vi "UMLEditor Main.vi"(1 "StartProject":string, 3 "StartTarget":string) -> ()   [LabVIEW 2020]
doc: "Main Open UML Modeller VI"
uses:
  <resource>/Framework/Providers/Open_GDS/UML/UMLEditor/UMLEditor statesType.ctl
  <resource>/Framework/Providers/Open_GDS/UML/UMLEditor/UMLEditor LocalVariablesType.ctl
  <resource>/Framework/Providers/Open_GDS/UML/Graphics_class/Graphics.lvclass
  <resource>/Framework/Providers/Open_GDS/UML/Grid_class/Grid.lvclass
  <resource>/Framework/Providers/Open_GDS/UML/UMLEditor/UMLEditor tooltype.ctl
  <resource>/Framework/Providers/Open_GDS/UML/UMLEditor/UMLEditor_DiagramInfo.ctl
  <resource>/Framework/Providers/Open_GDS/UML/Graph_class/Graph.lvclass
  <resource>/Framework/Providers/Open_GDS/UML/General/Point/Point Point2D.ctl
  <resource>/Framework/Providers/Open_GDS/UML/General/Rectangle/Rectangle Rectangle2D.ctl
  <resource>/Framework/Providers/Open_GDS/UML/AbstractEdge_class/AbstractEdge.lvclass
  <resource>/Framework/Providers/Open_GDS/UML/UMLEditor/UMLEditor ExportType.ctl
  <resource>/Framework/Providers/Open_GDS/UML/UMLEditor/UMLEditor FlattenCommandType.ctl
  <resource>/Framework/Providers/Open_GDS/UML/UMLEditor/UMLEditor ExecuteCommandType.ctl
  <resource>/Framework/Providers/Open_GDS/UML/ContextHelp/ContextHelp_EventType.ctl
  <resource>/Framework/Providers/Open_GDS/UML/AbstractNode_class/AbstractNode.lvclass
  <resource>/Framework/Providers/Open_GDS/UML/UMLEditor/UMLEditor_HotSpotData.ctl
  <resource>/Framework/Providers/Open_GDS/UML/UMLEditor/UMLEditor_HotSpotType.ctl
  <resource>/Framework/Providers/Open_GDS/UML/UmlEditor_class/EventData.ctl
  <resource>/Framework/Providers/Open_GDS/UML/ClassDiagramGraph_class/ClassDiagramGraph.lvclass
  C:/Program Files (x86)/National Instruments/LabVIEW 2020/resource/Framework/Providers/Open_GDS/UML/Graph_class/Graph.lvclass
  <resource>/Framework/Providers/Open_GDS/UML/DqmhModuleDiagramGraph_class/DqmhModuleDiagramGraph.lvclass
  <resource>/Framework/Providers/Open_GDS/UML/SequenceDiagramGraph_class/SequenceDiagramGraph.lvclass
  <resource>/Framework/Providers/Open_GDS/UML/StateDiagramGraph_class/StateDiagramGraph.lvclass
  <resource>/Framework/Providers/Open_GDS/UML/UseCaseDiagramGraph_class/UseCaseDiagramGraph.lvclass
  <resource>/Framework/Providers/Open_GDS/UML/UMLEditor/UMLEditor_Cursortype.ctl
  <resource>/Framework/Providers/Open_GDS/UML/UMLEditor/UMLEditor MenuActionType.ctl
  <resource>/Framework/Providers/Open_GDS/UML/Graphics_class/LvFontType.ctl
  <resource>/Framework/Providers/Open_GDS/UML/Graphics_class/FontType.ctl
  <resource>/Framework/Providers/Open_GDS/UML/UMLEditor/UMLEditor BusyDialogAction.ctl
  <resource>/Framework/Providers/Open_GDS/UML/UMLEditor/UMLEditor_StoredPathes.ctl
  <resource>/Framework/Providers/Open_GDS/ClassProviders/Common/File/File_StoredPathesActions.ctl
  <resource>/Framework/Providers/Open_GDS/UML/ContextHelp/ContextHelp_HelpTexts.ctl
  <resource>/Framework/Providers/Open_GDS/UML/GeneralPathEdge_class/GeneralPathEdge.lvclass
  C:/Program Files (x86)/National Instruments/LabVIEW 2020/resource/Framework/Providers/Open_GDS/UML/AbstractEdge_class/AbstractEdge.lvclass
  <resource>/Framework/Providers/Open_GDS/UML/ClassNode_class/ClassNode.lvclass
  C:/Program Files (x86)/National Instruments/LabVIEW 2020/resource/Framework/Providers/Open_GDS/UML/AbstractNode_class/AbstractNode.lvclass
  <vilib>/event_ctls.llb/eventvkey.ctl
  <resource>/Framework/Providers/Open_GDS/UML/Graph_class/SaveTypes.ctl
  <resource>/Framework/Providers/Open_GDS/UML/UMLEditor/UMLEditor_DiagramType.ctl
  <resource>/Framework/Providers/Open_GDS/UML/ClassNode_class/ExternalSetTypes.ctl
  <resource>/Framework/Providers/Open_GDS/UML/StateDiagramGraph_class/private/StateDiagramData.ctl
  <resource>/Framework/Providers/Open_GDS/UML/StateDiagramGraph_class/private/ViPathShowOption.ctl
  <resource>/Framework/Providers/Open_GDS/UML/UMLEditor/UMLEditor ClipBoardActionType.ctl
  <resource>/Framework/Providers/Open_GDS/UML/RectangularNode_class/RectangularNode.lvclass
  <resource>/Framework/Providers/Open_GDS/UML/ReversedEngineering/private/ReversedEngineering SyncUmlFromCodeActions.ctl
  <resource>/Framework/Providers/Open_GDS/ClassProviders/Common/CommonVIs/CommonVIs_StereoType.ctl
  Instance           1 22Saved   UMLEditor Main .vi
  Instance           2 22Saved   UMLEditor Main .vi
  <resource>/Framework/Providers/Open_GDS/ClassProviders/Provider_BaseClassInterface/ClassReader_class/ClassReader.lvclass
  <resource>/Framework/Providers/Open_GDS/UML/UMLEditor/UMLEditor ToolButtonsAction.ctl
  <resource>/Framework/Providers/Open_GDS/UML/UmlEditor_class/UmlEditor.lvclass
  <vilib>/Utility/cursorutil.llb/Set Cursor (Icon Pict).vi
panel:
  in  "GraphButtons":T1(radio)=enum."2" caption="Radio Buttons"
  out "SearchString":string caption="Search"
  in  "open":bool
  in  "close":bool
  in  "Diagram":u16(ring) items=["Class Diagram: 22.uml"]
  out "ProductPicture":picture
  out "Time":i32=21
  out "PictureMenuEvent":string
  out "RevHistory":bool
  in  "Help":bool
  in  "DragAndDropPath":path
  in  "ClassAggregationDialog":T2
  out "Picture":picture
  out "error out":errorcluster
  in  "Project":u16(ring) items=["GDS_Example_022.lvproj"]
  in  "Help":bool=TRUE
  in  "Target":u16(ring) items=["My Computer"]
  out "StatusBar":string
  in  "Sync":bool
  # "Class aggregation"
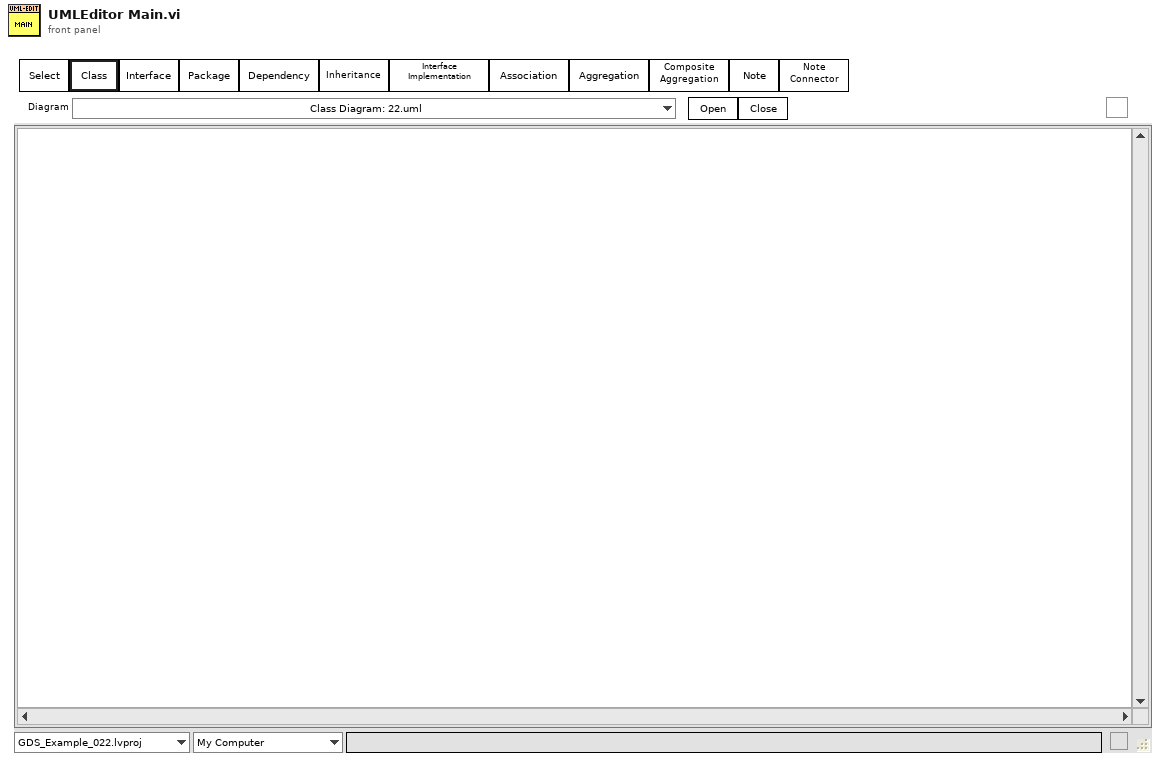
[diagram p1: front panel]
types:
  T1 = enum32{"1", "2", "3", "4", "5", "6", "7", "8", "9", "10", "11", "12", "13"}
  T2 = cluster{"AddAttribute":bool, "Don'tAddAttribute":bool, "Close":bool, "Text":string}
  T3 = typedef "UMLEditor MenuActionType.ctl" = enum16{"EnableSave", "EnablePaste", "DisablePaste", "DiableSave", "AddRecentFile", "disablePropDel", "enablePropDel", "enablePropDisDel", "diasbleClassRel", "enableClassRel", "Class", "State", "Other", "EnableXMI", "DisableXMI", "EnableCopy", "DisableCopy"}
  T4 = typedef "UMLEditor_Cursortype.ctl" = enum16{"Arrow", "Move", "Finger", "Wait", "NS", "WE", "NESW", "NWSE"}
  T5 = typedef "UMLEditor LocalVariablesType.ctl" = cluster{"state":T6, "graphics":refnum<class "Graphics.lvclass">, "grid":refnum<class "Grid.lvclass">, "toolType":T7, "diagramIndex":i32, "diagrams":T8[], "zoom":dbl, "hideGrid":bool, "lastMousePoint":T9, "rubberBandStart":T9, "dragStartPoint":T9, "dragStartBounds":T10, "gridColor":u32, "gridSize":dbl, "CONNECT_THRESHOLD":i32, "selected":T7, "selectedEdge":refnum<class "AbstractEdge.lvclass">, "butDwn":bool, "lastPress":u32, "modified":bool, "offset":T9, "menu":refnum<k9>, "file":path, "saveAs":bool, "newSelected":bool, "exportype":T11, "quit":bool, "revHistory":cluster{"rev":string, "text":string}[], "FlattenCommandSettings":T12, "PopUpMessageEvent":T14, "ResizePanelInProgress":bool, "NodesBounds":T10, "ToolHelp":bool, "ViRef":refnum<vi>, "FP_CtrlEnterEvents":refnum<event-registration>, "SelectedNodes":refnum<class "AbstractNode.lvclass">[], "mouse":refnum<k1>, "RevPlugInPath":path, "Action":string, "KeyPressTime":u32, "ObjectHotspots":T15[], "HotSpotCursor":bool, "HotSpotFunction":T16, "Don'tDeleteChildren":bool, "ShiftDown":bool, "CtrlDown":bool, "HotSpotNode":refnum<class "AbstractNode.lvclass">, "Sync":bool, "SyncTime":u32, "ForceSyncNow":bool, "LastSync":timestamp, "XMI_Import":bool, "Event":refnum<event-registration>}
  T6 = typedef "UMLEditor statesType.ctl" = enum16{"Idle", "CheckLicense", "revHistory", "Init", "Init2", "EditSelected", "RemoveSelected", "PaintComponent", "ChangeZoom", "ChangeGridSize", "Open", "Close", "Save", "ExportPicture", "Export", "Repaint", "Error", "Exit", "QUIT", "CreateScript", "ExecuteScript", "ClassReversedEngineering", "PlugInReverseEngineering", "StateReversedEngineering", "AutoPlace", "ExecuteCommand", "OpenClass", "SyncAll", "StraightenAssociation", "Copy", "Paste", "AddNodeFromProjectTree", "AddNodeFromProjectTree+SyncAll", "PanAndRepaint", "Init3", "CopyPaste", "ApplyDesignPattern", "AnalyseViInStateDiagram", "AutoSync"}
  T7 = typedef "UMLEditor tooltype.ctl" = enum16{"None", "Node", "Edge"}
  T8 = typedef "UMLEditor_DiagramInfo.ctl" = cluster{"name":string, "diagramType":string, "unsaved":bool, "graph":refnum<class "Graph.lvclass">, "saveDir":path}
  T9 = typedef "Point Point2D.ctl" = cluster{"x":dbl, "y":dbl}
  T10 = typedef "Rectangle Rectangle2D.ctl" = cluster{"x":dbl, "y":dbl, "width":dbl, "height":dbl}
  T11 = typedef "UMLEditor ExportType.ctl" = enum16{"None", "Printer", "png", "jpg", "roseUML"}
  T12 = typedef "UMLEditor FlattenCommandType.ctl" = cluster{"Command":T13, "CommandData":variant}
  T13 = typedef "UMLEditor ExecuteCommandType.ctl" = enum16{"SyncUmlFromCode", "SyncCodeFromUML", "OpenClass", "OpenFile", "CreateClass", "CreateVI", "OpenClassAttribute", "LocateInProject", "GraphExecute"}
  T14 = typedef "ContextHelp_EventType.ctl" = refnum<user-event>
  T15 = typedef "UMLEditor_HotSpotData.ctl" = cluster{"Node":refnum<class "AbstractNode.lvclass">, "HotSpot":T9, "Function":T16}
  T16 = typedef "UMLEditor_HotSpotType.ctl" = enum16{"N", "NE", "E", "SE", "S", "SW", "W", "NW", "Expand", "Collaps"}
  T17 = typedef "UMLEditor ToolButtonsAction.ctl" = enum16{"SelectSelect", "SetReferneces"}
  T18 = typedef "Graphics.lvclass/FontType.ctl" = cluster{"Font Name:":string, "Size":i16, "Strikeout?":bool, "Italic?":bool, "Underline?":bool, "Outline?":bool, "Shadow?":bool, "Bold?":bool}
  T19 = enum16{"CreateAggregation", "DeleteAggregation", "SetReferneces", "HideCluster", "GetStatus"}
  T20 = typedef "Graphics.lvclass/LvFontType.ctl" = enum16{"User-specified Font", "Application Font", "System Font", "Dialog Font"}
  T21 = typedef "UMLEditor_StoredPathes.ctl" = enum16{"LastSearchPath", "QueuedArrayStateVI", "ClassBasePath", "ViTemplatePath", "ApplicationTemplatePath", "IniFilePath", "WizDir", "RevPlugInPath"}
  T22 = typedef "UMLEditor BusyDialogAction.ctl" = enum16{"Initialize", "Open(VIs)", "Open(i)", "Send_I-Value", "SendStatusMessage", "GetBusyDialogStatus", "Close", "Quit"}
  T23 = enum16{"SetPopUpEventTask", "GetStatus", "SetOpenState", "SetDialogCaller", "SetToolHelp"}
  T24 = typedef "File_StoredPathesActions.ctl" = enum16{"Get Path", "Set Path", "Delete Path", "Clear All Paths"}
  T25 = typedef "ContextHelp_HelpTexts.ctl" = enum16{"None(Hide)", "Default", "Help", "Welcome", "GettingStarted", "ClassDiagram_Help", "SequenceDiagram_Help", "UseCaseDiagram_Help", "BSelect", "BClass", "BInterface", "BPackage", "BNote", "BDependency", "BInheritance", "BInterfaceImplementation", "BAssociation", "BAggregation", "BCompAggregation", "BNoteConnector", "BObject", "BActionBar", "BCall", "BSystem", "BActor", "BUseCase", "BGeneralization", "BIncludes", "BExtends", "BUseCaseDiagramAssociation", "ClassRelationshipEdge editDialog_Bent Style", "ClassRelationshipEdge editDialog_RelationType", "ClassRelationshipEdge editDialog_Reverse association", "ClassRelationshipEdge editDialog_Start label", "ClassRelationshipEdge editDialog_Middle label", "ClassRelationshipEdge editDialog_End label", "UMLEditor reversedEngineering_Pathes", "ReversedEngineering StateReverseDialog_Help", "ReversedEngineering StateQueuedSettings_Help", "UMLEditor reversedEngineering_AddTopVIs", "UMLEditor reversedEngineering_AddClasses", "UMLEditor reversedEngineering_AddDirs", "UMLEditor reversedEngineering_Recursively", "UMLEditor reversedEngineering_Remove", "UMLEditor reversedEngineering_ClearList", "UMLEditor reversedEngineering_HideSubAss", "UMLEditor reversedEngineering_CreateTypes", "UMLEditor reversedEngineering_OnlyInheritance", "UMLEditor reversedEngineering_CreateApplication", "UMLEditor reversedEngineering_OK", "UMLEditor reversedEngineering_Cancel", "UMLEditor reversedEngineering_Help", "UMLEditor createWizardScriptFile_ScriptfilePath", "UMLEditor createWizardScriptFile_ClassPath", "UMLEditor createWizardScriptFile_Use", "UMLEditor createWizardScriptFile_PrivateDirName", "UMLEditor createWizardScriptFile_DirAppend", "UMLEditor createWizardScriptFile_Separator Character", "UMLEditor createWizardScriptFile_OK", "UMLEditor createWizardScriptFile_Cancel", "UMLEditor createWizardScriptFile_Help", "ClassNode editDialog_Class Name", "InterfaceNode editDialog_Class Name", "ClassNode editDialog_Attribute", "ClassNode editDialog_Methods", "InterfaceNode editDialog_Methods", "ClassNode editDialog_connection", "InterfaceNode editDialog_connection", "ClassNode editDialog_StereoType", "ClassNode editDialog_ShowAttrib", "ClassNode editDialog_ShowMethods", "ClassNode editDialog_ClassPath", "ClassNode editDialog_AddAttribute", "ClassNode editDialog_AddMethod", "InterfaceNode editDialog_AddMethod", "ClassNode AttributeGuide_AttributeName", "ClassNode AttributeGuide_Array?", "ClassNode AttributeGuide_Data Type", "ClassNode AttributeGuide_RefName", "ClassNode AttributeGuide_Preview", "ClassNode AttributeGuide_OK", "ClassNode AttributeGuide_Cancel", "ClassNode MethodGuide_Visibility", "ClassNode MethodGuide_Method Name", "ClassNode MethodGuide_Preview", "ClassNode MethodGuide_OK", "ClassNode MethodGuide_Cancel", "CallNode EditCallProperties_AllButtons", "ObjectNode EditObjectlProperties_AllButtons", "ActorNode EditActorProperties_AllButtons", "UseCaseRelationshipNode EditUseCaselProperties_AllButtons", "UseCaseNode EditUseCaselProperties_AllButtons", "SystemNode EditSystemProperties_AllButtons", "ReversedEngineering UpdateAttributes_AllButtons", "StateNode editDialog_AllButtons", "StateTransition editDialog_AllButtons", "ArrangeNodes Main_Picture", "ArrangeNodes Main_Zoom", "ArrangeNodes Main_Auto Zoom", "ArrangeNodes Main_shorten", "ArrangeNodes Main_Min Length", "ArrangeNodes Main_Max Length", "ArrangeNodes Main_increase", "ArrangeNodes Main_decrease", "ArrangeNodes Main_Shake", "ArrangeNodes Main", "BState", "BInitialState", "BFinalState", "BStateTransition", "StateDiagram_Help", "StateDiagram_PropertiesAllButtons", "ReversedEngineering StateReverseDialog_ClearStates", "ReversedEngineering StateReverseDialog_UseQueuedStateMachines", "ReversedEngineering StateReverseDialog_QueuedSettings", "ReversedEngineering StateReverseDialog_SearchForVIs", "ReversedEngineering StateReverseDialog_SearchCriteria", "OptionsDialog_ClassBasePath", "OptionsDialog_VIPath", "OptionsDialog_ApplicationPath", "OptionsDialog_WizDir", "OptionsDialog_IniFilePath", "OptionsDialog_DefineColors", "OptionsDialog_Help", "OptionsDialog_CreateTypes", "ClassRelationshipEdge editDialog_SplitWire"}
  T26 = typedef "Graph.lvclass/SaveTypes.ctl" = enum16{"Normal", "XMI"}
  T27 = typedef "UMLEditor_DiagramType.ctl" = string
  T28 = typedef "ClassNode.lvclass/ExternalSetTypes.ctl" = enum16{"Name", "Attributes", "Methods", "Position", "ShowMethods", "ShowAttributes", "ClassPath"}
  T29 = typedef "StateDiagramGraph.lvclass/StateDiagramData.ctl" = cluster{"VI-Path":path, "ShowOption":T30}
  T30 = typedef "StateDiagramGraph.lvclass/ViPathShowOption.ctl" = enum16{"Don't Show", "Show Relative Path", "Show Absolute Path"}
  T31 = typedef "UMLEditor ClipBoardActionType.ctl" = enum16{"Init", "EmptyClipBoard", "InsertToClipBoard", "PasteContentAtPos"}
  T32 = enum16{"Left Button", "Center Button", "Right Button", "Window Close"}
  T33 = typedef "ReversedEngineering SyncUmlFromCodeActions.ctl" = enum16{"GetAttributes&MethodsFromCode", "GetAll"}
  T34 = typedef "CommonVIs_StereoType.ctl" = enum16{"None", "TYPE", "ENUM", "ABSTRACT", "ACTOR", "GUI", "SINGLETON", "SIGNAL", "BOUNDARY", "ENTITY", "CONTROL", "LEGACY", "APPLICATION", "VI", "LVLIB", "INTERFACE"}
  T35 = enum8{"Enabled", "Disabled", "Disabled and Grayed Out"}
  T36 = typedef "Graph.lvclass/ToolbarButtonType.ctl" = cluster{"Text":string, "Type":T7}
  T37 = cluster{"startNode":refnum<class "AbstractNode.lvclass">, "endNode":refnum<class "AbstractNode.lvclass">}
  T38 = typedef "ContextHelp_ShowType.ctl" = cluster{"Header":string, "Picture":picture, "Text":string}
  T39 = typedef "LVPoint32TypeDef.ctl" = cluster{"Horizontal":i32, "Vertical":i32}
  T40 = typedef "eventsource.ctl" = u32
  T41 = typedef "LVMouseTypeDef.ctl" = cluster{"Mouse Position":cluster{"X":i32, "Y":i32}, "Mouse Modifiers":cluster{"Button Down":bool, "Shift Mod":bool, "Menu Mod":bool, "Option Mod":bool}}
  T42 = typedef "LVBoundsTypeDef.ctl" = cluster{"Width":u32, "Height":u32}
  T43 = typedef "LVPointTypeDef.ctl" = cluster{"Horizontal":i16, "Vertical":i16}
  T44 = typedef "UMLEditor toolsType.ctl" = enum16{"CD_Select", "CD_Class", "CD_Interface", "CD_Package", "CD_Note", "CD_Dependency", "CD_Inheritance", "CD_InterfaceImp", "CD_Association", "CD_Aggregation", "CD_Composite", "CD_NoteConn", "SQD_Select", "SQD_Object", "SQD_ActionBar", "SQD_Note", "SQD_Call", "SQD_NoteConn", "UD_Select", "UD_System", "UD_Actor", "UD_UseCase", "UD_Note", "UD_Assoiciation", "UD_Generalization", "UD_GeneralizationIncludes", "UD_GeneralizationExtends", "UD_Realization", "UD_Relationship", "UD_NoteEdge", "STD_Select", "STD_State", "STD_InitailState", "STD_FinalState", "STD_ChoiseState", "STD_StateTransation", "STD_Note", "STD_NoteEdge", "DM_Select", "DM_VI", "DM_Module", "DM_Request", "DM_RequestWait", "DM_Roundtrip", "DM_Broadcast", "DM_Note", "DM_NoteEdge"}
  T45 = cluster{"Shift":bool, "Ctrl":bool, "Alt":bool, "Cmd":bool, "Opt":bool}
  T46 = typedef "UMLEditor EditorActionType.ctl" = enum16{"NoAction", "Repaint", "ExecuteCommand"}
  T47 = typedef "eventvkey.ctl" = enum16{"ASCII", "Enter", "Return", "Shift", "Ctrl", "Alt", "Cmd", "Opt", "Caps", "NumLock", "Clear", "Break", "Up", "Down", "Left", "Right", "Insert", "Delete", "Home", "End", "PageUp", "PageDown", "Escape", "Help", "Pause", "ScrollLock", "F1", "F2", "F3", "F4", "F5", "F6", "F7", "F8", "F9", "F10", "F11", "F12", "F13", "F14", "F15", "F16", "F17", "F18", "F19", "F20", "F21", "F22", "F23", "F24", "Play", "VolumeUp", "VolumeDown", "Mute", "Two Byte Char"}
  T48 = typedef "lveventtype.ctl" = enum32{"Null", "Timeout", "Annotation Menu Selection", "Annotation Menu Selection?", "App Instance Close", "App Instance Close?", "Autoscale Range Change", "Bookmark Info Change", "Cell Edit", "Cell Edit?", "Cursor Grab", "Cursor Grab?", "Cursor Menu Selection", "Cursor Menu Selection?", "Cursor Move", "Cursor Release", "Data Change", "Direction Change", "Display State Change", "Drag Ended", "Drag Enter", "Drag Leave", "Drag Over", "Drag Source Update", "Drag Starting", "Drag Starting?", "Drop", "Exec State Change", "Key Down", "Key Down?", "Key Repeat", "Key Repeat?", "Key Up", "Listbox Double Click", "Menu Activation?", "Menu Selection (App)", "Menu Selection? (App)", "Menu Selection (User)", "Mouse Down", "Mouse Down?", "Mouse Enter", "Mouse Leave", "Mouse Move", "Mouse Up", "Mouse Wheel", "NI Security User Change (App)", "Pane Size", "Panel Close", "Panel Close?", "Panel Resize", "Plot Attribute Change", "Scale Range Change", "Shortcut Menu Activation?", "Shortcut Menu Selection (App)", "Shortcut Menu Selection? (App)", "Shortcut Menu Selection (User)", "Tree Double Click", "Tree Drag", "Tree Drag?", "Tree Drop", "Tree Drop?", "Tree Item Close", "Tree Item Close?", "Tree Item Open", "Tree Item Open?", "User Event", "Value Change"}
  T49 = enum32{"existing file", "new file", "new or existing file", "existing dir", "new dir", "new or existing dir", "existing file (use LLBs)", "new file (use LLBs)", "new or existing file (use LLBs)", "new or existing file or directory (use LLBs)"}
  T50 = cluster{"button 1":bool, "button 2":bool, "button 3":bool, "button 4":bool}
  T51 = cluster{"Horizontal":i32, "Vertical":i32, "Scrolling":i32}
  T52 = typedef "LVRectTypeDef.ctl" = cluster{"Left":i16, "Top":i16, "Right":i16, "Bottom":i16}
  T53 = enum32{"Invalid", "Standard", "Closed", "Hidden", "Minimized", "Maximized"}
  T54 = typedef "AbstractNode.lvclass/NodeConnectionStatsType.ctl" = enum16{"NA", "Connect", "DisConnect"}
  T55 = typedef "Librarian File Info Out.ctl" = cluster{"creation date":u32, "last mod date":u32, "type":string, "creator":string, "LV version":i32, "size":i32, "top level":bool}
  T56 = typedef "Graph.lvclass/diagramType.ctl" = enum16{"None", "Class", "Sequency", "State", "UseCase"}
  T57 = typedef "DesignPatterns_Node.ctl" = cluster{"ID":string, "Type":T58, "Name":string, "Stereotype":string, "X":i32, "Y":i32, "TypeSpecificData":variant}
  T58 = typedef "DesignPatterns_NodeType.ctl" = enum16{"Class", "Interface", "Note", "Package"}
  T59 = typedef "DesignPatterns_Link.ctl" = cluster{"ID":string, "Type":T60, "Name":string, "StartText":string, "EndText":string, "From":string, "To":string, "BendStyle":string, "StartOffset":i32, "EndOffset":i32}
  T60 = typedef "DesignPatterns_LinkType.ctl" = enum16{"Dependency", "Inheritance", "Interface", "Association", "Aggregation", "CompositeAggregation"}
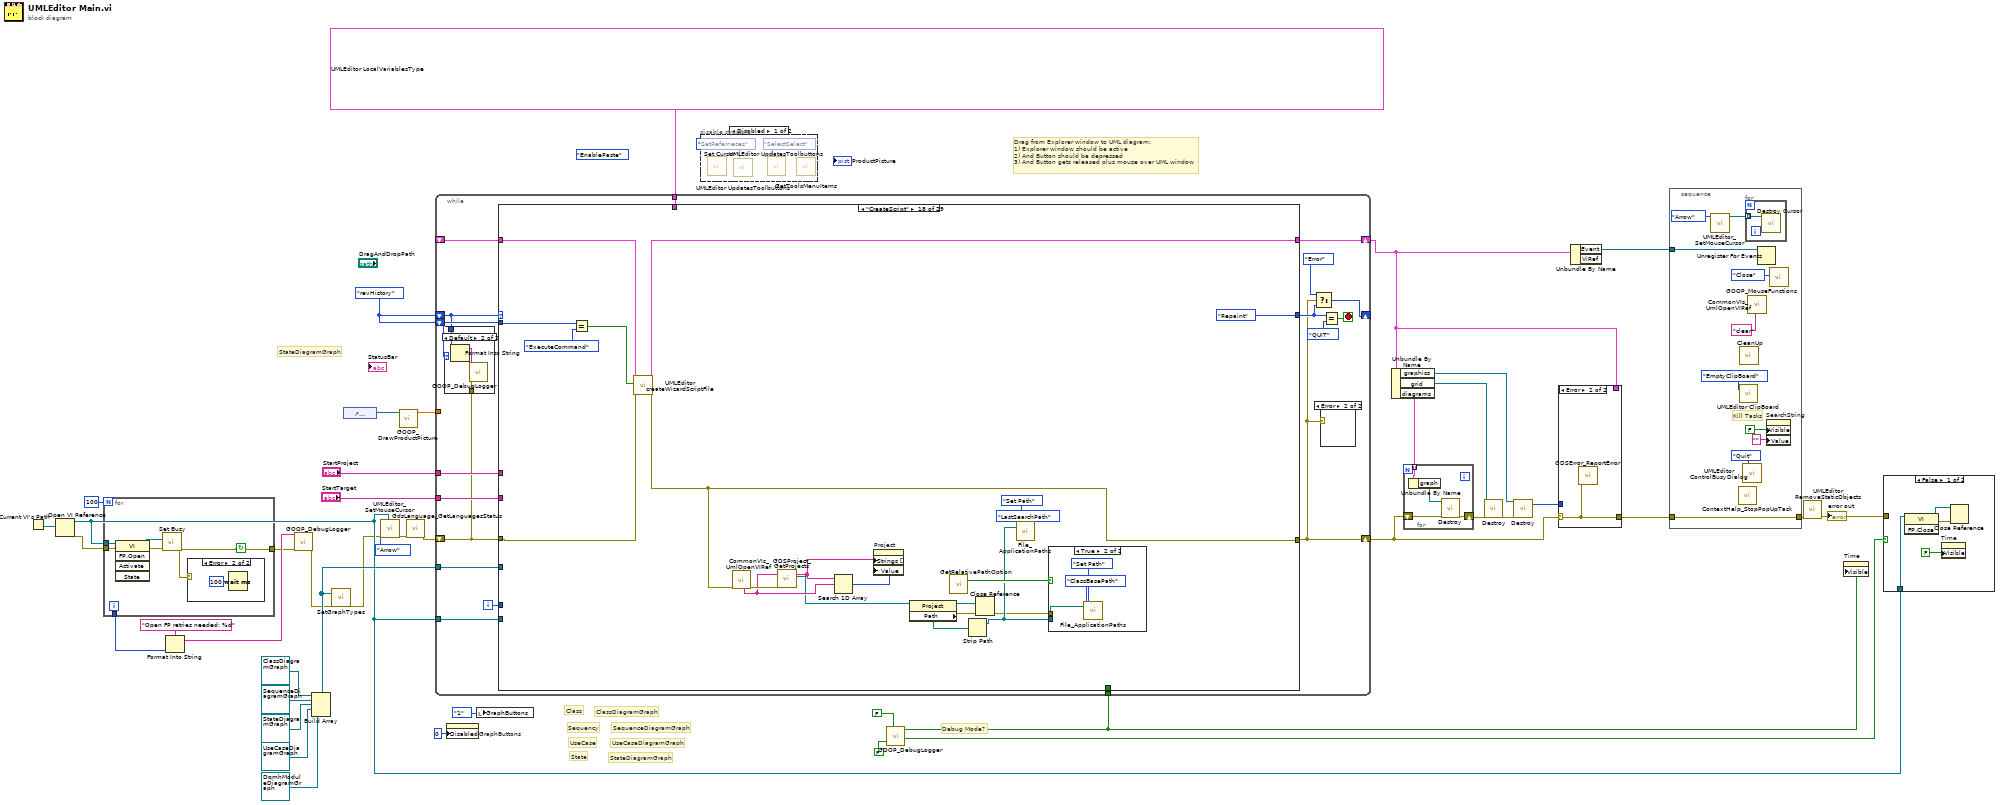
[diagram p0: block diagram]
diagram:
  (unwired) UMLEditor_MenuActionType."EnablePaste" ("menuAction")
  w37 = UMLEditor_statesType."revHistory" ("state")
  # "StateDiagramGraph"
  # "SequenceDiagramGraph"
  # "UseCaseDiagramGraph"
  # "State"
  # "UseCase"
  # "Sequency"
  # "ClassDiagramGraph"
  # "Class"
  # "StateDiagramGraph"
  # "Debug Mode?"
  # "Drag from Explorer window to UML diagram:\n1) Explorer window should be active\n2) And Button should be depressed\n3) And Button gets released plus mouse over UML window"
  n1 = Current VI's Path() -> (path=w34:path)
  n2 = Open VI Reference(vi path=w34) -> (vi reference=w9:refnum<vi>, error out=w8:errorcluster)  [unwired: 1 in, 4 out]
  n3 = for {
    N: 100 -> [_]
    tunnel: w9 -> [w49]
    tunnel: w8 -> [w48]
    tunnel: [w45] -> w3
    tunnel: [w44] -> w6
    i -> [w44]
    stop <- w45 continue-if-true
    n4 = invoke class="VI" method="FP.Open"(reference=w49, error in=w48) -> (reference out=w46:refnum<vi>, error out=w47:errorcluster)  [unwired: 3 in, 3 out]
    n5 = call <vilib>:"Set Busy.vi"("error in (no error)"=w47, "VI reference (current VI)"=w46) -> ("error out"=w45:errorcluster)  [unwired: 8 in, 1 out]
    n6 = case shown="Error" w45 {
      frame No Error {
      }
      frame Error {
        n7 = Wait (ms)(milliseconds to wait=u32 100) -> ()  [unwired: 1 out]
      }
    }
  }
  n8 = Format Into String(format string="Open FP retries needed: %d", w6) -> (resulting string=w4:string)  [unwired: 2 in, 1 out]
  n9 = call <resource>:"GOOP_DebugLogger.vi"("error in (no error)"=w3, "State"=w4) -> ("error out"=w2:errorcluster)  [unwired: 7 in, 2 out]
  n10 = Build Array(refnum<class "ClassDiagramGraph.lvclass"> refnum ("ClassDiagramGraph.lvclass"), refnum<class "SequenceDiagramGraph.lvclass"> refnum ("SequenceDiagramGraph.lvclass"), refnum<class "StateDiagramGraph.lvclass"> refnum ("StateDiagramGraph.lvclass"), refnum<class "UseCaseDiagramGraph.lvclass"> refnum ("UseCaseDiagramGraph.lvclass"), refnum<class "DqmhModuleDiagramGraph.lvclass"> refnum ("DqmhModuleDiagramGraph")) -> (w15:refnum<class "Graph.lvclass">[])
  n11 = call <resource>:"SetGraphTypes.vi"("GraphTypes"=w15, "error in (no error)"=w2) -> ("error out"=w1:errorcluster)  [unwired: 17 in]
  n12 = control-ref of="ProductPicture"() -> (w27:refnum<vi>)
  n13 = call <resource>:"UMLEditor_SetMouseCursor.vi"("ViRefToActOn"=w9, "error in (no error)"=w1, "CursorType"=UMLEditor_Cursortype."Arrow") -> ("error out"=w14:errorcluster)  [unwired: 7 in, 1 out]
  n14 = call <resource>:"GOOP_DrawProductPicture.vi"("ProductPictureControl"=w27) -> ("Zoom Factor"=w26:sgl)  [unwired: 10 in]
  n15 = call <resource>:"GdsLanguage_GetLanguagesStatus.vi"("error in (no error)"=w14) -> ("error out"=w32:errorcluster)  [unwired: 18 out]
  n16 = property on="GraphButtons" class="RadioBtnsControl (strict)"("Disabled"=u8 0) -> ()  [unwired: 2 in, 2 out]
  n17 = local write "GraphButtons"(T1."1" ("GraphButtons")) -> ()
  n18 = disable-structure shown="Disabled" {
    frame Disabled {
      n19 = call-poly <vilib>:"Set Cursor.vi"() -> ()  [unwired: 10 in, 2 out]
      n20 = call <resource>:"UMLEditor UpdatesToolbuttons.vi"("Action(SelectSelect)"=UMLEditor_ToolButtonsAction."SetReferneces") -> ()  [unwired: 5 in, 14 out]
      n21 = call <resource>:"UMLEditor UpdatesToolbuttons.vi"("Action(SelectSelect)"=UMLEditor_ToolButtonsAction."SelectSelect") -> ()  [unwired: 5 in, 14 out]
      n22 = call-dynamic "GetToolsMenuItems.vi"() -> ()  [unwired: 17 in, 3 out]
    }
    frame Enabled {
    }
  }
  n23 = call <resource>:"GOOP_DebugLogger.vi"("ActivateDon'tCloseVI"=FALSE ("ActivateDebugging"), "ActivateDebugging"=FALSE) -> ("Don'tCloseVI"=w24:bool, "Debugging"=w25:bool)  [unwired: 7 in, 1 out]
  n24 = while {
    shift-right: [w53] -> _
    shift-left: w37 -> [w58]
    shift-right: [w60] -> w28
    shift-left: w32 -> [w55]
    shift-right: [w67] -> w31
    shift-left: _ -> [w66]
    tunnel: T5 {"state"=enum."Idle", "graphics"=refnum, "grid"=refnum, "toolType"=enum."None", "diagramIndex"=0, "diagrams"=[], "zoom"=0.0, "hideGrid"=FALSE, "lastMousePoint"={"x"=0.0, "y"=0.0}, "rubberBandStart"={"x"=0.0, "y"=0.0}, "dragStartPoint"={"x"=0.0, "y"=0.0}, "dragStartBounds"={"x"=0.0, "y"=0.0, "width"=0.0, "height"=0.0}, "gridColor"=0, "gridSize"=0.0, "CONNECT_THRESHOLD"=0, "selected"=enum."None", "selectedEdge"=refnum, "butDwn"=FALSE, "lastPress"=0, "modified"=FALSE, "offset"={"x"=0.0, "y"=0.0}, "menu"=refnum, "file"=path "", "saveAs"=FALSE, "newSelected"=FALSE, "exportype"=enum."None", "quit"=FALSE, "revHistory"=[], "FlattenCommandSettings"={"Command"=enum."SyncUmlFromCode", "CommandData"=variant}, "PopUpMessageEvent"=refnum, "ResizePanelInProgress"=FALSE, "NodesBounds"={"x"=0.0, "y"=0.0, "width"=0.0, "height"=0.0}, "ToolHelp"=FALSE, "ViRef"=refnum, "FP_CtrlEnterEvents"=refnum, "SelectedNodes"=[], "mouse"=refnum, "RevPlugInPath"=path "", "Action"="", "KeyPressTime"=0, "ObjectHotspots"=[], "HotSpotCursor"=FALSE, "HotSpotFunction"=enum."N", "Don'tDeleteChildren"=FALSE, "ShiftDown"=FALSE, "CtrlDown"=FALSE, "HotSpotNode"=refnum, "Sync"=FALSE, "SyncTime"=0, "ForceSyncNow"=FALSE, "LastSync"=timestamp(0 s since 1904-01-01), "XMI_Import"=FALSE, "Event"=refnum} ("localVariables") -> [w68]
    shift-left: w37 -> [w64]
    tunnel: "StartProject" -> [w62]
    tunnel: w25 -> [w61]
    tunnel: "StartTarget" -> [w59]
    tunnel: w26 -> [_]
    tunnel: w15 -> [w57]
    tunnel: w9 -> [w56]
    i -> [w63]
    stop <- w70 stop-if-true
    n25 = case shown="Default" w58 {
      tunnel: w58 -> [_ w73]
      tunnel: w55 -> [_ w71]
      frame "Idle", "PaintComponent", "Repaint" {
      }
      frame Default {
        n26 = Format Into String(w73) -> (resulting string=w72:string)  [unwired: 3 in, 1 out]
        n27 = call <resource>:"GOOP_DebugLogger.vi"("error in (no error)"=w71, "State"=w72) -> ()  [unwired: 7 in, 3 out]
      }
    }
    n28 = case shown="\"CreateScript\"" w58 {
      selector: w58 -> [_ _ _ _ _ w260 _ w3396 _ w3655 _ _ _ _ _ _ _ _ w4310 _ _ _ _ _ _ _ _ _ _]
      tunnel: [UMLEditor_statesType."CheckLicense" ("state") w81 UMLEditor_statesType."Init2" ("state") UMLEditor_statesType."Init3" ("state") w243 w255 w3311 w3407 w3601 w3662 UMLEditor_statesType."Repaint" ("state") UMLEditor_statesType."Idle" ("state") UMLEditor_statesType."Repaint" ("state") UMLEditor_statesType."Repaint" ("state") w3995 w4100 w4216 UMLEditor_statesType."Repaint" ("state") w4311 UMLEditor_statesType."Repaint" ("state") w4481 UMLEditor_statesType."Idle" ("state") UMLEditor_statesType."Repaint" ("state") w4745 UMLEditor_statesType."Repaint" ("state") UMLEditor_statesType."Repaint" ("state") UMLEditor_statesType."Repaint" ("state") w5261 w5288] -> w65
      tunnel: w55 -> [w75 w80 w92 w215 w241 w265 w3310 w3416 w3593 w3659 w3683 w3753 w3804 w3938 w4013 w4115 w4220 w4304 w4317 w4445 w4484 w4549 w4721 w4741 w5104 w5160 w5239 w5251 w5278]
      tunnel: [w75 w84 w145 w200 w241 w266 w3310 w3409 w3603 w3658 w3687 w3744 w3806 w3931 w4012 w4090 w4222 w4284 w4316 w4434 w4472 w4518 w4720 w4744 w5105 w5148 w5227 w5262 w5284] -> w60
      tunnel: w68 -> [w78 _ _ _ _ _ _ _ _ _ _ _ _ _ _ _ _ _ _ _ _ _ _ _ _ _ _ _ _]
      tunnel: [w77 w79 w139 w219 w242 w262 w3306 w3410 w3602 w3656 w3678 w3724 w3800 w3928 w4009 w4105 w4215 w4301 w4313 w4450 w4474 w4524 w4718 w4738 w5103 w5151 w5235 w5255 w5279] -> w67
      tunnel: w66 -> [_ w79 w147 w196 w242 w256 w3295 w3401 w3589 w3656 w3679 w3724 w3796 w3934 w3992 w4098 w4212 w4302 w4309 w4450 w4474 w4528 w4719 w4735 w5102 w5137 w5231 w5250 w5279]
      tunnel: w64 -> [_ w89 _ _ _ _ _ _ _ _ _ _ _ _ w3998 _ w4214 w4303 _ _ _ w4540 _ _ _ w5142 _ _ w5281]
      tunnel: w63 -> [_ _ _ _ _ _ _ _ _ _ _ _ _ _ _ _ _ _ _ _ _ _ _ _ _ _ _ _ _]
      tunnel: w62 -> [_ _ _ w208 _ _ _ _ _ _ _ _ _ _ _ _ _ _ _ _ _ _ _ _ _ _ _ _ _]
      tunnel: w61 -> [_ _ _ _ _ _ _ _ _ _ _ _ _ _ _ _ _ _ _ _ _ w4517 _ _ _ _ _ _ _]
      tunnel: w59 -> [_ _ _ w187 _ _ _ _ _ _ _ _ _ _ _ _ _ _ _ _ _ _ _ _ _ _ _ _ _]
      tunnel: w57 -> [_ _ w93 _ _ _ _ _ _ _ _ _ _ _ _ _ _ _ _ _ _ _ _ _ _ _ _ _ _]
      tunnel: w56 -> [_ _ _ w183 w240 _ _ _ _ _ _ _ _ _ _ _ _ _ _ _ _ _ _ _ _ _ _ _ _]
      frame "revHistory" {
        n29 = Bundle By Name(cluster=w78, "revHistory"=cluster{"rev":string, "text":string}[] []) -> (w77:T5)
      }
      frame "CheckLicense" {
        n30 = Equal?(x=w89, y=UMLEditor_statesType."Idle" ("state")) -> (x = y?=w85:bool)
        n31 = Current VI's Menubar() -> (w83:refnum<k9>)
        n32 = call <resource>:"UMLEditor menuUpdates.vi"("menu"=w83, "menuAction"=UMLEditor_MenuActionType."EnableXMI", "error in (no error)"=w80) -> ("error out"=w84:errorcluster)  [unwired: 3 in, 13 out]
        n33 = Select(t=UMLEditor_statesType."Idle" ("state"), s=w85, f=UMLEditor_statesType."Init" ("state")) -> (s? t:f=w81:T6)
      }
      frame "Init" {
        w169 = T9 {"x"=nan, "y"=nan} ("lastMousePoint")
        w126 = 10.0  # gridSize
        w144 = 0 ("offsetX")
        w116 = FALSE ("Help")
        w146 = "Untitled 1" ("name")
        w127 = u32 14803425
        n34 = control-ref of="Picture"() -> (w124:refnum<vi>)
        n35 = control-ref of="GraphButtons"() -> (w109:refnum<vi>)
        n36 = property on="ClassAggregationDialog" class="Clust (strict)"("Visible"=FALSE) -> ()  [unwired: 2 in, 2 out]
        n37 = property on="Picture" class="Pict"("Visible"=TRUE) -> ()  [unwired: 2 in, 2 out]
        n38 = control-ref of="AddAttribute"() -> (w130:refnum<vi>)
        n39 = control-ref of="Don'tAddAttribute"() -> (w129:refnum<vi>)
        n40 = control-ref of="ClassAggregationDialog"() -> (w125:refnum<vi>)
        n41 = control-ref of="Text"() -> (w128:refnum<vi>)
        n42 = property class="RadioBtnsControl (strict)"(reference=w109) -> ("Controls[]"=w108:refnum<vi>[])  [unwired: 1 in, 2 out]
        n43 = call <resource>:"Init.vi"("GraphButtons"=w109, "error in (no error)"=w92) -> ("Event"=w110:refnum<user-event>, "error out"=w135:errorcluster)  [unwired: 16 out]
        n44 = register-events(error in=w135, w110, w108) -> (reference out=w134:refnum<event-registration>, error out=w118:errorcluster)  [unwired: 1 in]
        n45 = call <resource>:"Graphics_Create.vi"("screenRef"=w124, "error in (no error)"=w118) -> ("reference out"=w161:refnum<class "Graphics.lvclass">, "error out"=w160:errorcluster)  [unwired: 1 in, 15 out]
        n46 = call <resource>:"setFont.vi"("reference"=w161, "fontType"=LvFontType."User-specified Font", "font"=T18 {"Font Name:"="Arial", "Size"=14, "Strikeout?"=FALSE, "Italic?"=FALSE, "Underline?"=FALSE, "Outline?"=FALSE, "Shadow?"=FALSE, "Bold?"=FALSE}, "error in (no error)"=w160) -> ("reference out"=w159:refnum<class "Graphics.lvclass">, "error out"=w158:errorcluster)  [unwired: 14 out]
        n47 = call <resource>:"getScreenBounds.vi"("reference"=w159, "error in (no error)"=w158) -> ("reference out"=w175:refnum<class "Graphics.lvclass">, "bounds"=w150:T10, "error out"=w181:errorcluster)  [unwired: 15 out]
        n48 = call <resource>:"Grid_Create.vi"("gridColor"=w127, "error in (no error)"=w181) -> ("reference out"=w178:refnum<class "Grid.lvclass">, "error out"=w179:errorcluster)  [unwired: 1 in, 15 out]
        n49 = call <resource>:"setGrid.vi"("reference"=w178, "gridX"=w126, "gridY"=w126, "error in (no error)"=w179) -> ("reference out"=w177:refnum<class "Grid.lvclass">, "error out"=w180:errorcluster)  [unwired: 14 out]
        n50 = call <resource>:"UMLEditor_AggregationClusterDialogControl.vi"("OK-Button"=w130, "Cancel-Button"=w129, "String"=w128, "Cluster"=w125, "Action(SelectSelect)"=T19."SetReferneces", "screenRef"=w124) -> ()  [unwired: 3 in, 11 out]
        n51 = call-dynamic "draw.vi"("reference"=w177, "graphics"=w175, "bounds"=w150, "error in (no error)"=w180) -> ("reference out"=w176:refnum<class "Grid.lvclass">, "error out"=w142:errorcluster)  [unwired: 14 in]
        n52 = call <resource>:"updateScreen.vi"("reference"=w175, "error in (no error)"=w142) -> ("reference out"=w174:refnum<class "Graphics.lvclass">, "picture"=w90:picture, "error out"=w137:errorcluster)  [unwired: 15 out]
        n53 = local write "Picture"(w90) -> ()
        n54 = call <resource>:"UMLEditor_IniFilePath.vi"("error in (no error)"=w137) -> ("Get Path"=w138:path, "error out"=w136:errorcluster)  [unwired: 1 in, 16 out]
        n55 = Current VI's Menubar() -> (w95:refnum<k9>)
        n56 = call <resource>:"UMLEditor loadIniFileInfo.vi"("menu"=w95, "iniFile"=w138, "error in (no error)"=w136) -> ("StabilityProblems"=w115:bool, "SyncTime"=w117:u32, "Ini-FileFound"=w140:bool, "ToolHelp"=w141:bool, "LastDiagramType"=w107:T27, "FileToOpen"=w119:path, "error out"=w106:errorcluster)  [unwired: 10 out]
        n57 = call <resource>:"CreateGraphFromName.vi"("GraphTypeToCreate"=w107, "error in (no error)"=w106) -> ("GraphCreated"=w104:refnum<class "Graph.lvclass">, "error out"=w105:errorcluster)  [unwired: 16 in]
        n58 = local write "GraphButtons"(T1."1" ("GraphButtons")) -> ()
        n59 = call-dynamic "GetGraphTypeInfo.vi"("reference in"=w104, "error in (no error)"=w105) -> ("reference out"=w102:refnum<class "Graph.lvclass">, "GraphTypeName"=w103:string, "error out"=w101:errorcluster)  [unwired: 12 in, 3 out]
        n60 = property on="Diagram" class="Ring (strict)"("Tip Strip"=w146) -> ()  [unwired: 2 in, 2 out]
        n61 = case shown="False" w140 {
          frame False {
            n62 = call <resource>:"UMLEditor GettingStartedDialog.vi"() -> ()  [unwired: 1 out]
          }
          frame True {
          }
        }
        n63 = call-dynamic "GetToolbarButtons.vi"("reference"=w102, "error in (no error)"=w101) -> ("reference out"=w100:refnum<class "Graph.lvclass">, "AllToolbarButtons"=w112:T36[], "error out"=w99:errorcluster)  [unwired: 13 in, 2 out]
        n64 = call <resource>:"UpdateToolbar.vi"("ToolbarButtons"=w112, "error in (no error)"=w99) -> ("error out"=w98:errorcluster)  [unwired: 17 in]
        n65 = Unbundle By Name(w147) -> ("diagrams"=w165:T8[])
        n66 = call <resource>:"UMLEditor ToolsMenuUpdates.vi"("menu"=w95, "Graph"=w100, "error in (no error)"=w98) -> ("error out"=w91:errorcluster)  [unwired: 2 in, 14 out]
        n67 = Index Array(array=w165) -> (element=w164:T8)  [unwired: 1 in]
        n68 = Bundle By Name(cluster=w164, "name"=w146, "diagramType"=w103, "unsaved"=FALSE, "graph"=w100, "saveDir"=path "") -> (w152:T8)
        n69 = call <resource>:"GOOP_MouseFunctions.vi"("error in (no error)"=w91, "StabilityProblem"=w115, "Action(Read)"=enum16{"Init", "Read", "Close"}."Init") -> ("error out"=w96:errorcluster)  [unwired: 6 in, 2 out]
        n70 = Build Array(w152) -> (w162:T8[])
        n71 = local write "Help"(w116) -> ()
        n72 = Set Menu Item Info(7:"Undo" ("item tag"), 9:FALSE ("enabled"), 11:w95) -> ()  [unwired: 1 in, 5 out]
        n73 = call <resource>:"UMLEditor_GraphMemory.vi"("GraphIn"=w100) -> ()  [unwired: 1 in, 18 out]
        n74 = local write "Sync"(w116) -> ()
        n75 = call <resource>:"UMLEditor UpdateNewMenu.vi"("menu"=w95, "GraphTypes"=w93, "error in (no error)"=w96) -> ("error out"=w94:errorcluster)  [unwired: 16 in]
        n76 = Bundle By Name(cluster=w147, "Sync"=w116, "ToolHelp"=w141, "menu"=w95, "grid"=w176, "graphics"=w174, "toolType"=UMLEditor_tooltype."None", "diagramIndex"=0, "zoom"=1.0, "hideGrid"=FALSE, "lastMousePoint"=w169, "rubberBandStart"=w169, "dragStartPoint"=w169, "dragStartBounds"=T10 {"x"=nan, "y"=nan, "width"=nan, "height"=nan}, "gridColor"=w127, "gridSize"=w126, "CONNECT_THRESHOLD"=8, "selected"=UMLEditor_tooltype."None" ("selcted"), "diagrams"=w162, "offset"=T9 {"x"=0.0, "y"=0.0}, "Event"=w134, "file"=w119, "SyncTime"=w117) -> (w139:T5)
        n77 = call <resource>:"UMLEditor menuUpdates.vi"("menu"=w95, "menuAction"=UMLEditor_MenuActionType."DiableSave", "error in (no error)"=w94) -> ("error out"=w148:errorcluster)  [unwired: 3 in, 13 out]
        n78 = property on="GraphButtons" class="RadioBtnsControl (strict)"("Disabled"=u8 0) -> ()  [unwired: 2 in, 2 out]
        n79 = call <resource>:"UMLEditor updateDiagramsInfo.vi"("localVariables"=w139, "error in (no error)"=w148) -> ("diagramNames"=w154:string[], "index"=w153:i32, "error out"=w145:errorcluster)  [unwired: 15 out]
        n80 = property on="Picture" class="Pict"("Origin:Left"=w144, "Origin:Top"=w144) -> (error out=w114:errorcluster)  [unwired: 2 in, 1 out]
        n81 = local write "Diagram"(w153) -> ()
        n82 = property on="Diagram" class="Ring (strict)"("Strings []"=w154) -> ()  [unwired: 2 in, 2 out]
        n83 = property on="Picture" class="Pict"(error in=w114, "Cursor"=0) -> ()  [unwired: 1 in, 2 out]
        n84 = property on="SearchString" class="Str"("Visible"=FALSE, "Value"="" ("SearchString")) -> ()  [unwired: 2 in, 2 out]
      }
      frame "Init2" {
        n85 = call <resource>:"GDSProject_GetProjects.vi"("error in (no error)"=w215, "OpenProjectRef(True)"=FALSE) -> ("Projects"=w211:string[], "error out"=w213:errorcluster)  [unwired: 1 in, 15 out]
        n86 = local write "StatusBar"("" ("StatusBar")) -> ()
        n87 = Search 1D Array(1D array=w211, element=w208) -> (index of element=w210:i32)  [unwired: 1 out]
        n88 = Empty String/Path?(string/path=w187) -> (empty?=w189:bool)
        n89 = call <resource>:"File_ApplicationPaths.vi"("PathName"=UMLEditor_StoredPathes."WizDir" ("UMLPathes")) -> ()  [unwired: 3 in, 16 out]
        n90 = case shown="0, Default" w210 {
          selector: w210 -> [w225 _]
          tunnel: [w225 u8 0 ("t")] -> w209
          frame 0, Default {
          }
          frame -1 {
          }
        }
        n91 = Select(t="My Computer" ("element"), s=w189, f=w187) -> (s? t:f=w186:string)
        n92 = Index Array(array=w211, index=w209) -> (element=w214:string)
        n93 = Empty Array?(array=w211) -> (empty?=w212:bool)
        n94 = property on="Project" class="Ring (strict)"("Strings []"=w211, "Value"=w209) -> ()  [unwired: 2 in, 2 out]
        n95 = case shown="False" w212 {
          tunnel: w214 -> [w235 _]
          tunnel: w213 -> [w234 w239]
          tunnel: [w233 w239] -> w206
          tunnel: [w232 _] -> w191
          tunnel: [w231 _] -> w190
          tunnel: w186 -> [w230 _]
          frame False {
            n96 = call <resource>:"UMLEditor_TargetDialog.vi"("error in (no error)"=w234, "Target"=w230, "GetProjectRefByName"=w235) -> ("error out"=w233:errorcluster, "ProjectFolder"=w227:path, "TargetIndex"=w231:u16, "Targets"=w232:string[])  [unwired: 4 in, 1 out]
            n97 = call <resource>:"GetRelativePathOption.vi"() -> ("UseProjectFolderAsBasePath"=w229:bool)  [unwired: 1 in, 18 out]
            n98 = case shown="True" w229 {
              tunnel: w227 -> [_ w237]
              tunnel: File_StoredPathesActions."Set Path" ("Method (Get Path)") -> [_ w236]
              frame False {
              }
              frame True {
                n99 = call <resource>:"File_ApplicationPaths.vi"("PathName"=UMLEditor_StoredPathes."ClassBasePath" ("UMLPathes"), "Path In"=w237, "Method (Get Path)"=w236) -> ()  [unwired: 1 in, 16 out]
              }
            }
          }
          frame True {
          }
        }
        n100 = property on="Target" class="Ring (strict)"("Strings []"=w191, "Value"=w190) -> ()  [unwired: 2 in, 2 out]
        n101 = Unbundle By Name(w196) -> ("menu"=w199:refnum<k9>)
        n102 = call <resource>:"UMLEditor ControlBusyDialog.vi"("error in (no error)"=w206, "Action(SendStatusMessage)"=UMLEditor_BusyDialogAction."Initialize" ("Action")) -> ("error out"=w217:errorcluster)  [unwired: 2 in, 15 out]
        n103 = call <resource>:"GetToolTip.vi"("error in (no error)"=w206) -> ("ToolTip"=w205:cluster{"ToolTipOpen":bool, "LastToolTip":i32})  [unwired: 18 out]
        n104 = call <resource>:"UMLEditor AddToolsMenuItems.vi"("menu"=w199, "GoopWizExists"=FALSE, "error in (no error)"=w217) -> ("error out"=w184:errorcluster)  [unwired: 1 in, 15 out]
        n105 = Unbundle By Name(w205) -> ("ToolTipOpen"=w204:bool)
        n106 = Unbundle By Name(w196) -> ("ToolHelp"=w220:bool)
        n107 = call <resource>:"ContextHelp_StartPopUpTask.vi"("CallerRef"=w183, "error in (no error)"=w184) -> ("PopUpTaskEvent"=w218:T14, "error out"=w221:errorcluster)  [unwired: 16 out]
        n108 = case shown="True" w204 {
          frame False {
          }
          frame True {
            n109 = call <resource>:"ShowToolTips.vi"() -> ()  [unwired: 1 in, 19 out]
          }
        }
        n110 = call <resource>:"ContextHelp_Memory.vi"("State"=w220, "error in (no error)"=w221, "Actio(GetStatus)n"=T23."SetToolHelp") -> ("error out"=w198:errorcluster)  [unwired: 1 in, 15 out]
        n111 = call <resource>:"UMLEditor menuUpdates.vi"("menu"=w199, "menuAction"=UMLEditor_MenuActionType."disablePropDel") -> ()  [unwired: 4 in, 14 out]
        n112 = call <resource>:"UMLEditor getDiagramInfo.vi"("localVariables"=w196, "error in (no error)"=w198) -> ("graph"=w197:refnum<class "Graph.lvclass">, "error out"=w195:errorcluster)  [unwired: 16 out]
        n113 = Bundle By Name(cluster=w196, "ViRef"=w183, "PopUpMessageEvent"=w218) -> (w219:T5)
        n114 = call <resource>:"GetUndoOption.vi"("error in (no error)"=w195) -> ("UndoSize"=w193:i32, "error out"=w194:errorcluster)  [unwired: 17 out]
        n115 = call <resource>:"UndoEngine.vi"("Reference In"=w197, "Action"=enum16{"TakeSnapshot", "Undo", "Redo"}."TakeSnapshot", "Reset"=TRUE, "error in (no error)"=w194, "menu"=w199, "UndoLevels(ignoredIfNotWired)"=w193) -> ("error out"=w200:errorcluster)  [unwired: 2 in, 11 out]
      }
      frame "Init3" {
        n116 = call <vilib>:"Unset Busy.vi"("error in (no error)"=w241, "VI reference (current VI)"=w240) -> ()  [unwired: 9 in, 1 out]
        n117 = Unbundle By Name(w242) -> ("file"=w247:path)
        n118 = Empty String/Path?(string/path=w247) -> (empty?=w246:bool)
        n119 = Select(t=UMLEditor_statesType."Idle" ("state"), s=w246, f=UMLEditor_statesType."Open" ("state")) -> (s? t:f=w243:T6)
      }
      frame "Idle" {
        n120 = Unbundle By Name(w256) -> ("butDwn"=w267:bool, "Event"=w257:refnum<event-registration>)
        n121 = Bundle By Name(cluster=w256, "state"=w260) -> (w261:T5)
        n122 = call <resource>:"UMLEditor getDiagramInfo.vi"("localVariables"=w256, "error in (no error)"=w265) -> ("graph"=w263:refnum<class "Graph.lvclass">, "diagramType"=w259:T27, "error out"=w264:errorcluster)  [unwired: 15 out]
        n123 = event shown="[26] Menu Selection (User)" {
          selector: w257 -> [_ _ _ _ _ _ _ _ _ _ _ _ _ _ _ _ _ _ _ _ _ _ _ _ _ _ _ _ _ _]
          dyn-events: _ -> [_ _ _ _ _ _ _ _ _ _ _ _ _ _ _ _ _ _ _ _ _ _ _ _ _ _ _ _ _ _]
          timeout: 10 ("t") -> [_ _ _ _ _ _ _ _ _ _ _ _ _ _ _ _ _ _ _ _ _ _ _ _ _ _ _ _ _ _]
          tunnel: w267 -> [_ _ _ _ _ _ _ _ _ w414 _ _ _ _ _ _ _ _ _ _ _ _ _ _ _ _ _ _ _ w2705]
          tunnel: w261 -> [w277 w328 w334 w348 w381 w385 w393 w402 w407 w410 w865 w872 w875 w1206 w1269 w1358 w1539 w1673 w1737 w1759 w1768 w1812 w1826 w1845 w1951 w1954 w2245 w2692 w2698 w2704]
          tunnel: [w276 w329 w334 w350 w380 w385 w393 w403 w407 w420 w865 w873 w876 w1208 w1284 w1357 w1538 w1673 w1737 w1759 w1769 w1812 w1826 w1844 w1952 w1967 w2247 w2693 w2697 w2700] -> w262
          tunnel: w264 -> [w273 w321 w336 w370 w379 w387 w397 w401 w408 w418 w866 w874 w902 w1202 w1290 w1362 w1542 w1671 w1730 w1761 w1770 w1817 w1824 w1843 w1948 w1963 w2251 w2690 w2699 w2703]
          tunnel: [w278 w321 w335 w352 w377 w386 w396 w401 w408 w417 w866 w874 w897 w1201 w1279 w1364 w1544 w1674 w1731 w1760 w1770 w1816 w1823 w1842 w1948 w1964 w2250 w2690 w2699 w2702] -> w266
          tunnel: w263 -> [w275 _ _ _ w378 _ _ _ _ w421 _ _ w898 _ w1275 w1355 w1536 _ _ _ _ _ w1821 _ _ w1962 w2249 _ _ w2701]
          tunnel: w259 -> [_ _ w330 _ _ _ _ _ _ w419 _ _ _ _ _ _ _ _ _ _ _ _ _ _ _ w1961 w2248 _ _ _]
          tunnel: w256 -> [_ _ _ _ _ _ _ _ _ _ _ _ _ _ _ w1354 _ _ _ _ _ _ _ _ _ _ w2246 _ _ _]
          tunnel: [_ _ _ _ _ _ _ _ _ _ w863 _ _ _ _ _ _ _ _ _ _ _ _ _ _ _ _ _ _ _] -> _
          event "ClassAggregationDialog": Value Change {
            n124 = event-data() -> ()  [unwired: 7 out]
            n125 = Unbundle By Name("ClassAggregationDialog") -> ("AddAttribute"=w268:bool)  [unwired: 1 out]
            n126 = property on="ClassAggregationDialog" class="Clust (strict)"("Visible"=FALSE) -> ()  [unwired: 2 in, 2 out]
            n127 = call <resource>:"UMLEditor_AggregationClusterDialogControl.vi"("error in (no error)"=w273, "Action(SelectSelect)"=T19."GetStatus") -> ("StartEndNodes"=w270:T37, "AddAggregate?"=w271:bool, "error out"=w272:errorcluster)  [unwired: 7 in, 8 out]
            n128 = case shown="True" w268 {
              tunnel: w277 -> [w282 w292]
              tunnel: w272 -> [w283 w293]
              tunnel: [w283 w286] -> w278
              tunnel: [w282 w291] -> w276
              tunnel: w275 -> [_ w288]
              tunnel: w271 -> [_ w285]
              tunnel: w270 -> [_ w284]
              frame False {
              }
              frame True {
                n129 = case shown="False" w285 {
                  tunnel: w293 -> [w298 w304]
                  tunnel: w292 -> [w297 w305]
                  tunnel: [w296 w301] -> w290
                  tunnel: [w295 w302] -> w289
                  tunnel: [w294 w303] -> w287
                  tunnel: w284 -> [_ w300]
                  frame True {
                    n130 = Unbundle By Name(w297) -> ("selectedEdge"=w299:refnum<class "AbstractEdge.lvclass">)
                    n131 = call <resource>:"UMLEditor CreateAggregationAttributes.vi"("ClassAggregation"=w299, "error in (no error)"=w298) -> ("NodeModified"=w294:refnum<class "AbstractNode.lvclass">, "Modified?"=w296:bool, "error out"=w295:errorcluster)  [unwired: 15 out]
                  }
                  frame False {
                    n132 = Unbundle By Name(w305) -> ()  [unwired: 1 out]
                    n133 = call <resource>:"UMLEditor RemoveAggregationAttributes.vi"("StartEndNodes"=w300, "error in (no error)"=w304) -> ("NodeModified"=w303:refnum<class "AbstractNode.lvclass">, "Modified?"=w301:bool, "error out"=w302:errorcluster)  [unwired: 15 out]
                  }
                }
                n134 = case shown="True" w290 {
                  tunnel: w292 -> [w307 w317]
                  tunnel: [w307 w316] -> w291
                  tunnel: w289 -> [w306 w314]
                  tunnel: w288 -> [_ w313]
                  tunnel: w287 -> [_ w312]
                  tunnel: [w306 w309] -> w286
                  frame False {
                  }
                  frame True {
                    n135 = Build Array(w312) -> (w311:refnum<class "AbstractNode.lvclass">[])
                    n136 = call-dynamic "layout.vi"("reference"=w313, "LayoutNodes(Empty=All)"=w311, "error in (no error)"=w314) -> ("error out"=w310:errorcluster)  [unwired: 15 in, 1 out]
                    n137 = Bundle By Name(cluster=w317, "modified"=TRUE, "state"=UMLEditor_statesType."Repaint") -> (w308:T5)
                    n138 = call <resource>:"UMLEditor setDiagramInfo.vi"("error in (no error)"=w310, "localVariablesIn"=w308, "action"=enum16{"Name/Dir", "Unsaved", "Saved"}."Unsaved") -> ("localVariablesOut"=w316:T5, "error out"=w309:errorcluster)  [unwired: 2 in, 13 out]
                  }
                }
              }
            }
            n139 = stacked-sequence {
              tunnel: [T2 {"AddAttribute"=FALSE, "Don'tAddAttribute"=FALSE, "Close"=FALSE, "Text"=""} ("ClassAggregationDialog")] -> w269
              tunnel: w268 -> [_]
              frame #0 {
              }
            }
            n140 = local write "ClassAggregationDialog"(w269) -> ()
          }
          event "close": Value Change {
            n141 = event-data() -> ()  [unwired: 6 out]
            n142 = Unbundle By Name(w328) -> ("diagrams"=w327:T8[])
            n143 = Array Size(array=w327) -> (size(s)=w326:i32)
            n144 = Greater Than 0?(x=w326) -> (x > 0?=w325:bool)
            n145 = Select(t=UMLEditor_statesType."Close" ("state"), s=w325, f=UMLEditor_statesType."Idle" ("state")) -> (s? t:f=w323:T6)
            n146 = Bundle By Name(cluster=w328, "state"=w323, "selected"=UMLEditor_tooltype."None" ("selcted")) -> (w329:T5)
          }
          event "Diagram": Mouse Enter {
            n147 = event-data() -> ()  [unwired: 3 out]
            n148 = Unbundle By Name(w334) -> ("ToolHelp"=w333:bool)
            n149 = local read "Help"() -> (w332:bool)
            n150 = And(x=w333, y=w332) -> (x .and. y?=w331:bool)
            n151 = case shown="True" w331 {
              tunnel: w336 -> [w337 w341]
              tunnel: [w337 w340] -> w335
              tunnel: w334 -> [_ _]
              tunnel: w330 -> [_ w339]
              frame False {
              }
              frame True {
                n152 = case shown="\"StateDiagramGraph\"" w339 {
                  tunnel: [ContextHelp_HelpTexts."Default" ("HelpText") ContextHelp_HelpTexts."ClassDiagram_Help" ("HelpText") ContextHelp_HelpTexts."SequenceDiagram_Help" ("HelpText") ContextHelp_HelpTexts."UseCaseDiagram_Help" ("HelpText") ContextHelp_HelpTexts."StateDiagram_Help" ("HelpText")] -> w338
                  frame "None", Default {
                  }
                  frame "ClassDiagramGraph" {
                  }
                  frame "SequenceDiagramGraph" {
                  }
                  frame "UseCaseDiagramGraph" {
                  }
                  frame "StateDiagramGraph" {
                  }
                }
                n153 = call <resource>:"ContextHelp_HelpTexts.vi"("HelpText (enum or string)"=w338) -> ("HelpOut"=w342:T38)  [unwired: 18 out]
                n154 = call <resource>:"ContextHelp_SendMessageToPopUp.vi"("PopUpMessage"=w342, "error in (no error)"=w341) -> ("error out"=w340:errorcluster)  [unwired: 1 in, 16 out]
              }
            }
          }
          event "Diagram": Value Change {
            n155 = event-data() -> ()  [unwired: 2 out]
            n156 = Bundle By Name(cluster=w348, "state"=UMLEditor_statesType."Repaint", "diagramIndex"="Diagram", "toolType"=UMLEditor_tooltype."None", "selectedEdge"=refnum<class "AbstractEdge.lvclass"> refnum, "SelectedNodes"=refnum<class "AbstractNode.lvclass">[] []) -> (w350:T5)
            n157 = Unbundle By Name(w350) -> ("menu"=w356:refnum<k9>)
            n158 = call <resource>:"UMLEditor getDiagramInfo.vi"("localVariables"=w350, "error in (no error)"=w370) -> ("graph"=w358:refnum<class "Graph.lvclass">, "name"=w363:string, "saveDir"=w366:path, "error out"=w357:errorcluster)  [unwired: 14 out]
            n159 = Empty String/Path?(string/path=w366) -> (empty?=w365:bool)
            n160 = Build Path(base path=w366, name or relative path=w363) -> (appended path=w368:path)
